vi "ComputeBlocks.vi"(7 "SHA-1":refnum<class "SHA-1.lvclass">, 10 "blocks queue":refnum<queue>) -> (2 "hash":u8[](array[numeric]) format="%02x")   [LabVIEW 2013, in "SHA-1.lvlib" / "SHA-1.lvclass"]
doc: "This VI contains the core of the MD5 algorithm."
uses:
  SHA-1.lvclass
  Data-vector.ctl
  W-vector.ctl
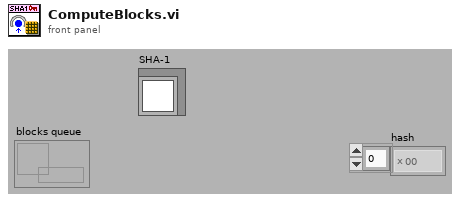
[diagram p1: front panel]
types:
  T1 = typedef "SHA-1.lvlib/SHA-1.lvclass/W-vector.ctl" = cluster{"W[ ]":u32[], "end":bool}
  T2 = typedef "SHA-1.lvlib/SHA-1.lvclass/Data-vector.ctl" = cluster{"Data[ ]":u8[], "end":bool}
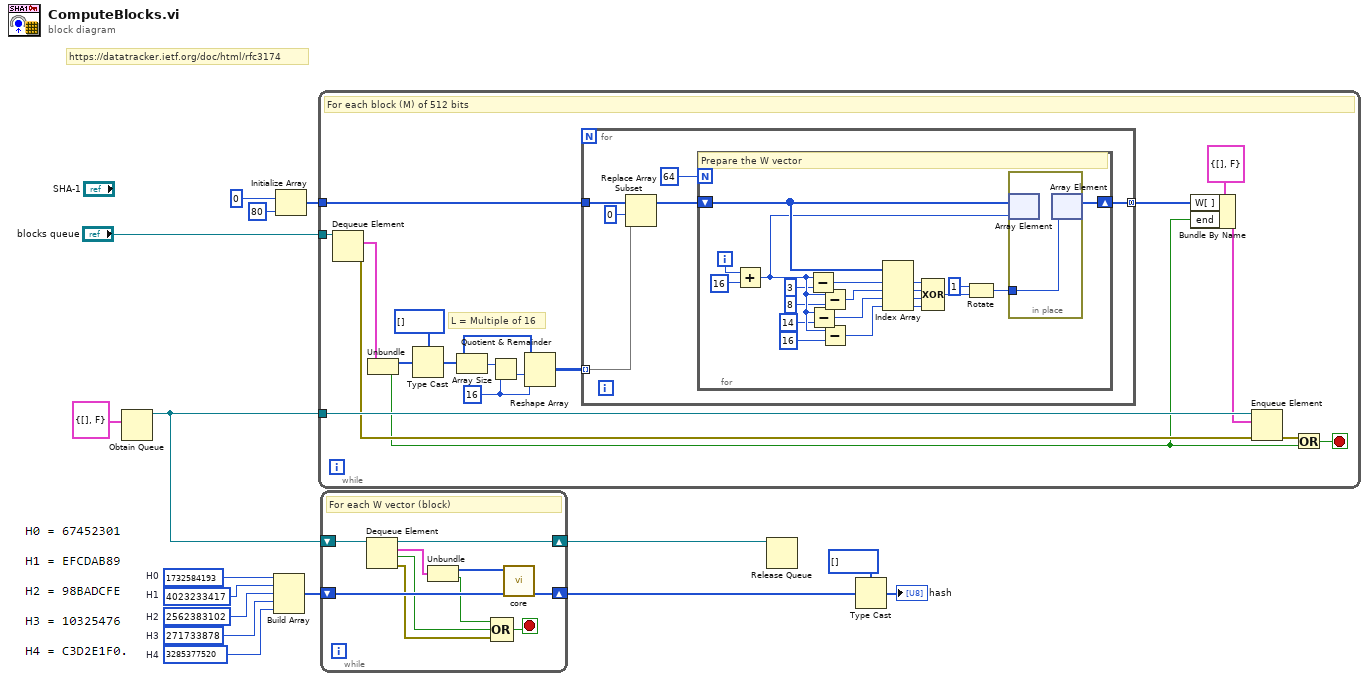
[diagram p0: block diagram]
diagram:
  w11 = u32 3285377520  # H4
  w12 = u32 271733878  # H3
  w13 = u32 2562383102  # H2
  w14 = u32 4023233417  # H1
  w15 = u32 1732584193  # H0
  # "https://datatracker.ietf.org/doc/html/rfc3174"
  n1 = Obtain Queue(element data type=T1 {"W[ ]"=[], "end"=FALSE} ("cluster")) -> (queue out=w8:refnum<queue>)  [unwired: 4 in, 2 out]
  n2 = Build Array(w15, w14, w13, w12, w11) -> (w3:u32[])
  n3 = Initialize Array(u32 0, 80) -> (w1:u32[])
  n4 = while {
    tunnel: "blocks queue" -> [w34]
    tunnel: w8 -> [w31]
    tunnel: w1 -> [w19]
    stop <- w18 stop-if-true
    w25 = 16 ("y")
    # "L = Multiple of 16"
    # "For each block (M) of 512 bits"
    n5 = Dequeue Element(queue=w34) -> (element=w33:T2, error out=w27:errorcluster)  [unwired: 2 in, 2 out]
    n6 = Unbundle(w33) -> ("Data[ ]"=w32:u8[], "end"=w17:bool)
    n7 = Type Cast(type=u32[] [] ("U32"), x=w32) -> (*(type *) &x=w22:u32[])
    n8 = Array Size(array=w22) -> (size(s)=w23:i32)
    n9 = Quotient & Remainder(x=w23, y=w25) -> (floor(x/y)=w24:i32)  [unwired: 1 out]
    n10 = Reshape Array(w22, w24, w25) -> (w21:u32[][])
    n11 = for {
      tunnel: w21 -> [w38] mode=indexing
      tunnel: [w36] -> w20 mode=concatenating
      tunnel: w19 -> [w35]
      n12 = Replace Array Subset(array=w35, new element=w38, index=0) -> (w37:u32[])
      n13 = for {
        N: 64 -> [_]
        shift-right: [w60] -> w36
        shift-left: w37 -> [w58]
        i -> [w56]
        # "Prepare the W vector"
        n14 = Add(x=w56, y=16) -> (x+y=w55:i32)
        n15 = Subtract(x=w55, y=3) -> (x-y=w46:i32)
        n16 = Subtract(x=w55, y=14) -> (x-y=w44:i32)
        n17 = Subtract(x=w55, y=8) -> (x-y=w45:i32)
        n18 = Subtract(x=w55, y=16) -> (x-y=w43:i32)
        n19 = Index Array(array=w58, index #1=w46, index #2=w45, index #3=w44, index #4=w43) -> (element #1=w50:u32, element #2=w49:u32, element #3=w48:u32, element #4=w47:u32)
        n20 = Compound Arithmetic op=XOR(w50, w49, w48, w47) -> (w41:u32)
        n21 = Rotate(1:w41, 2:i8 1 ("y")) -> (0:w59:u32)
        n22 = in-place {
          in-place-border: w59 -> [w61]
          n23 = in-place-array #1(w58, w55) -> ()  [unwired: 1 out]
          n24 = in-place-array #1(w61) -> (w60:u32[])  [unwired: 1 out]
        }
      }
    }
    n25 = Bundle By Name(cluster=T1 {"W[ ]"=[], "end"=FALSE}, "W[ ]"=w20, "end"=w17) -> (w28:T1)
    n26 = Enqueue Element(queue=w31, element=w28, error in (no error)=w27) -> (error out=w26:errorcluster)  [unwired: 1 in, 2 out]
    n27 = Or(x=w26, y=w17) -> (x .or. y?=w18:bool)
  }
  n28 = while {
    shift-right: [w70] -> w9
    shift-left: w3 -> [w71]
    shift-right: [w66] -> w4
    shift-left: w8 -> [w69]
    stop <- w62 stop-if-true
    # "For each W vector (block)"
    n29 = Dequeue Element(queue=w69) -> (queue out=w66:refnum<queue>, element=w68:T1, timed out?=w64:bool, error out=w63:errorcluster)  [unwired: 2 in]
    n30 = Unbundle(w68) -> ("W[ ]"=w67:u32[], "end"=w65:bool)
    n31 = Compound Arithmetic op=OR(w65, w64, w63) -> (w62:bool)
    n32 = call "core.vi"("H[5] in"=w71, "W[ ]"=w67) -> ("H[5] out"=w70:u32[])  [unwired: 9 in]
  }
  n33 = Release Queue(queue=w4) -> ()  [unwired: 2 in, 3 out]
  n34 = Type Cast(type=u8[] [], x=w9) -> (*(type *) &x=→"hash":u8[])
